vi "RemoteVI HTML Escape.vi"(0 "text":string) -> (4 "html":string)   [LabVIEW 2020, in "RemoteVI.lvlib"]
doc: "Text for HTML: & < > and \" written as their character references (the ampersand first). Pure function, cannot fail. Reference: htmlEscape() in tools\\lib\\server-app.mjs."
uses:
  RemoteVI.lvlib
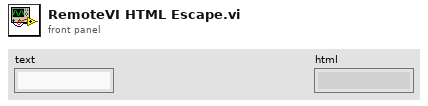
[diagram p1: front panel]
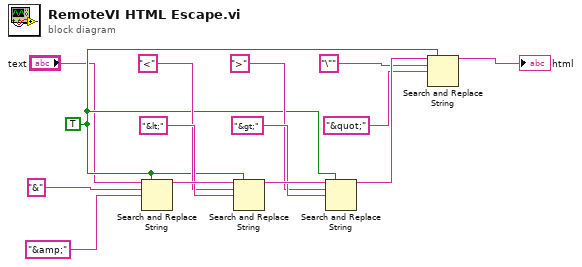
[diagram p0: block diagram]
diagram:
  w2 = TRUE
  n1 = Search and Replace String(replace all?=w2, input string="text", search string="&", replace string="&amp;") -> (result string=w11:string)  [unwired: 4 in, 3 out]
  n2 = Search and Replace String(replace all?=w2, input string=w11, search string="<", replace string="&lt;") -> (result string=w12:string)  [unwired: 4 in, 3 out]
  n3 = Search and Replace String(replace all?=w2, input string=w12, search string=">", replace string="&gt;") -> (result string=w13:string)  [unwired: 4 in, 3 out]
  n4 = Search and Replace String(replace all?=w2, input string=w13, search string="\"", replace string="&quot;") -> (result string=→"html":string)  [unwired: 4 in, 3 out]
